vi "Initialize Main Page.vi"(8 "error in (no error)":errorcluster, 10 "Main Page Controls":T2, 11 "Item Ref in":T1 format="%.0x") -> (0 "error out":errorcluster, 3 "Item Ref out":T1 format="%.0x")   [LabVIEW 2020, in "SLSC Switch System Explorer.lvlib"]
uses:
  SLSC Switch System Explorer.lvlib
  Main Page Controls.ctl
  <vilib>/NI VeriStand/Custom Device API/Custom Device Item Ref.ctl
  <vilib>/SLSC_Switch/Get Topologies (Simulate).vi
  Scripting/SLSC Switch Scripting.lvlib
  <vilib>/SLSC_Switch/SLSC Switch.lvlib
  <vilib>/NI VeriStand/Custom Device API/Custom Device API.lvlib
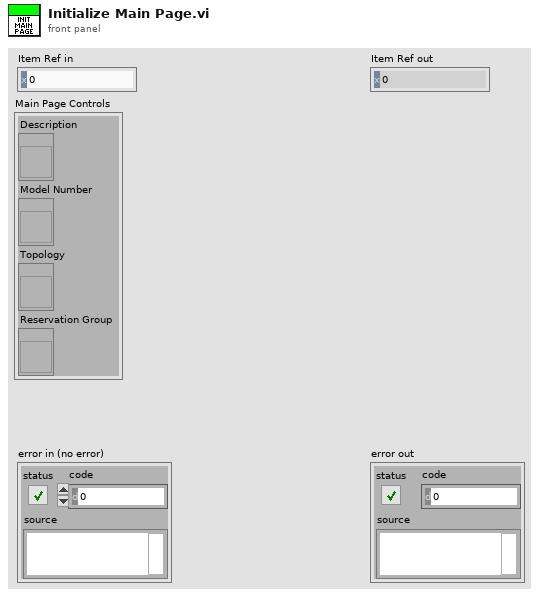
[diagram p1: front panel]
types:
  T1 = typedef "Custom Device API.lvlib/Custom Device Item Ref.ctl" = u64
  T2 = typedef "SLSC Switch System Explorer.lvlib/Main Page Controls.ctl" = cluster{"Description":refnum<vi>, "Model Number":refnum<vi>, "Topology":refnum<vi>, "Reservation Group":refnum<vi>}
  T3 = typedef "SLSC Switch Scripting.lvlib/SLSC Switch All Properties.ctl" = cluster{"Product Name":string, "Topology":string, "Switches JSON":string, "Description":string, "Reservation Group":string}
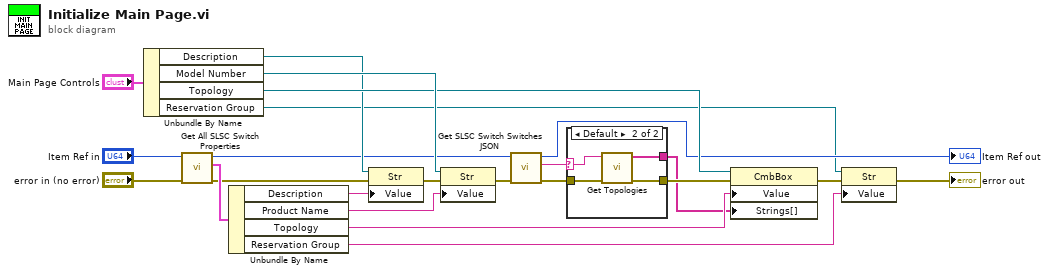
[diagram p0: block diagram]
diagram:
  n1 = Unbundle By Name("Main Page Controls") -> ("Description"=w16:refnum<vi>, "Model Number"=w22:refnum<vi>, "Topology"=w18:refnum<vi>, "Reservation Group"=w2:refnum<vi>)
  n2 = call "Get All SLSC Switch Properties.vi"("error in"="error in (no error)", "slsc switch custom device in"="Item Ref in") -> ("error out"=w12:errorcluster, "properties"=w21:T3, "slsc switch custom device out"=w9:T1)  [unwired: 7 in]
  n3 = Unbundle By Name(w21) -> ("Description"=w15:string, "Product Name"=w20:string, "Topology"=w19:string, "Reservation Group"=w1:string)
  n4 = property class="Str"(reference=w16, error in=w12, "Value"=w15) -> (error out=w17:errorcluster)  [unwired: 1 out]
  n5 = property class="Str"(reference=w22, error in=w17, "Value"=w20) -> (error out=w8:errorcluster)  [unwired: 1 out]
  n6 = call "Get SLSC Switch Switches JSON.vi"("error in"=w8, "slsc switch custom device in"=w9) -> ("error out"=w10:errorcluster, "switches json"=w11:string, "slsc switch custom device out"=→"Item Ref out":T1)  [unwired: 7 in]
  n7 = case shown="Default" w11 {
    selector: w11 -> [_ w28]
    tunnel: w10 -> [w24 w27]
    tunnel: [w24 w26] -> w7
    tunnel: [_ w25] -> w6
    frame "" {
    }
    frame Default {
      n8 = call-poly <vilib>:"Get Topologies.vi"("error in (no error)"=w27, "switches json"=w28) -> ("error out"=w26:errorcluster, "topologies"=w25:string[])  [unwired: 8 in]
    }
  }
  n9 = property class="CmbBox"(reference=w18, error in=w7, "Value"=w19, "Strings[]"=w6) -> (error out=w4:errorcluster)  [unwired: 1 out]
  n10 = property class="Str"(reference=w2, error in=w4, "Value"=w1) -> (error out=→"error out":errorcluster)  [unwired: 1 out]
